vi "4.Open_Select_Profile_Vi.vi"(8 "error in (no error)":errorcluster, 10 "Boolean":bool, 11 "VI Selection":T1=enum."Option window Vi") -> (0 "error out":errorcluster)   [LabVIEW 2021]
uses:
  Control/Vi_selection.ctl
panel:
  out "error in (no error) 2":errorcluster
  out "element":path
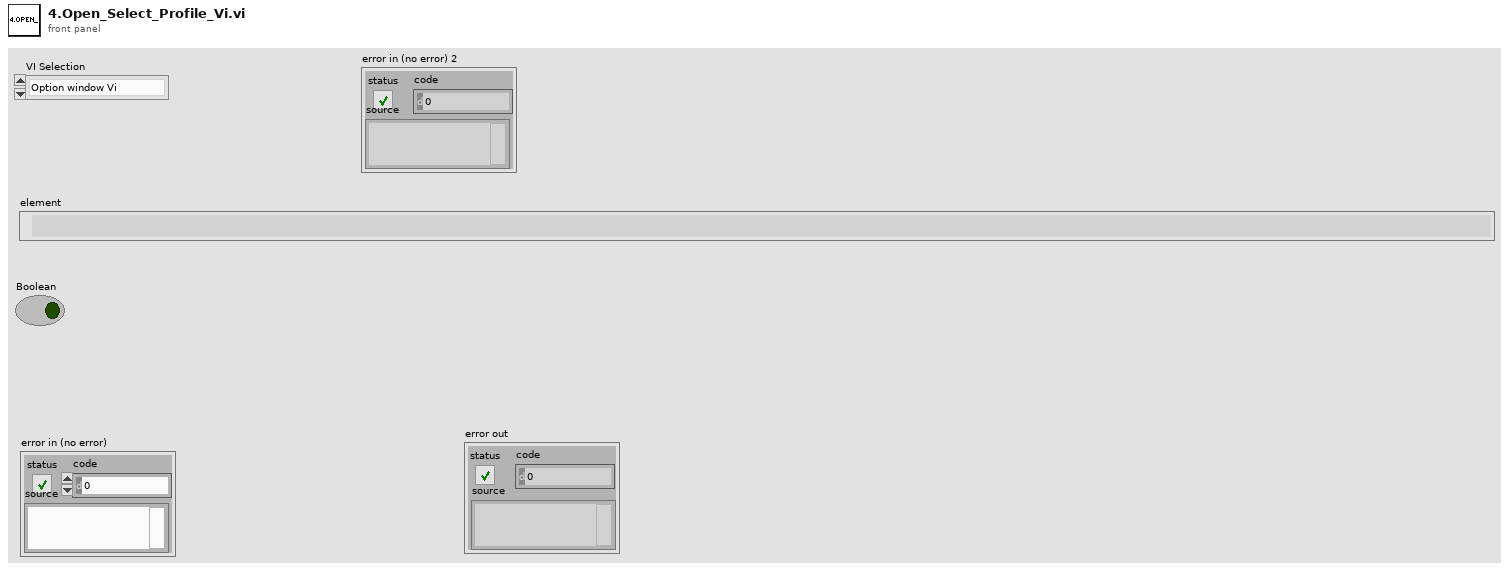
[diagram p1: front panel]
types:
  T1 = typedef "Vi_selection.ctl" = enum16{"Test Editor", "Option window Vi"}
  T2 = enum32{"Invalid", "Standard", "Closed", "Hidden", "Minimized", "Maximized"}
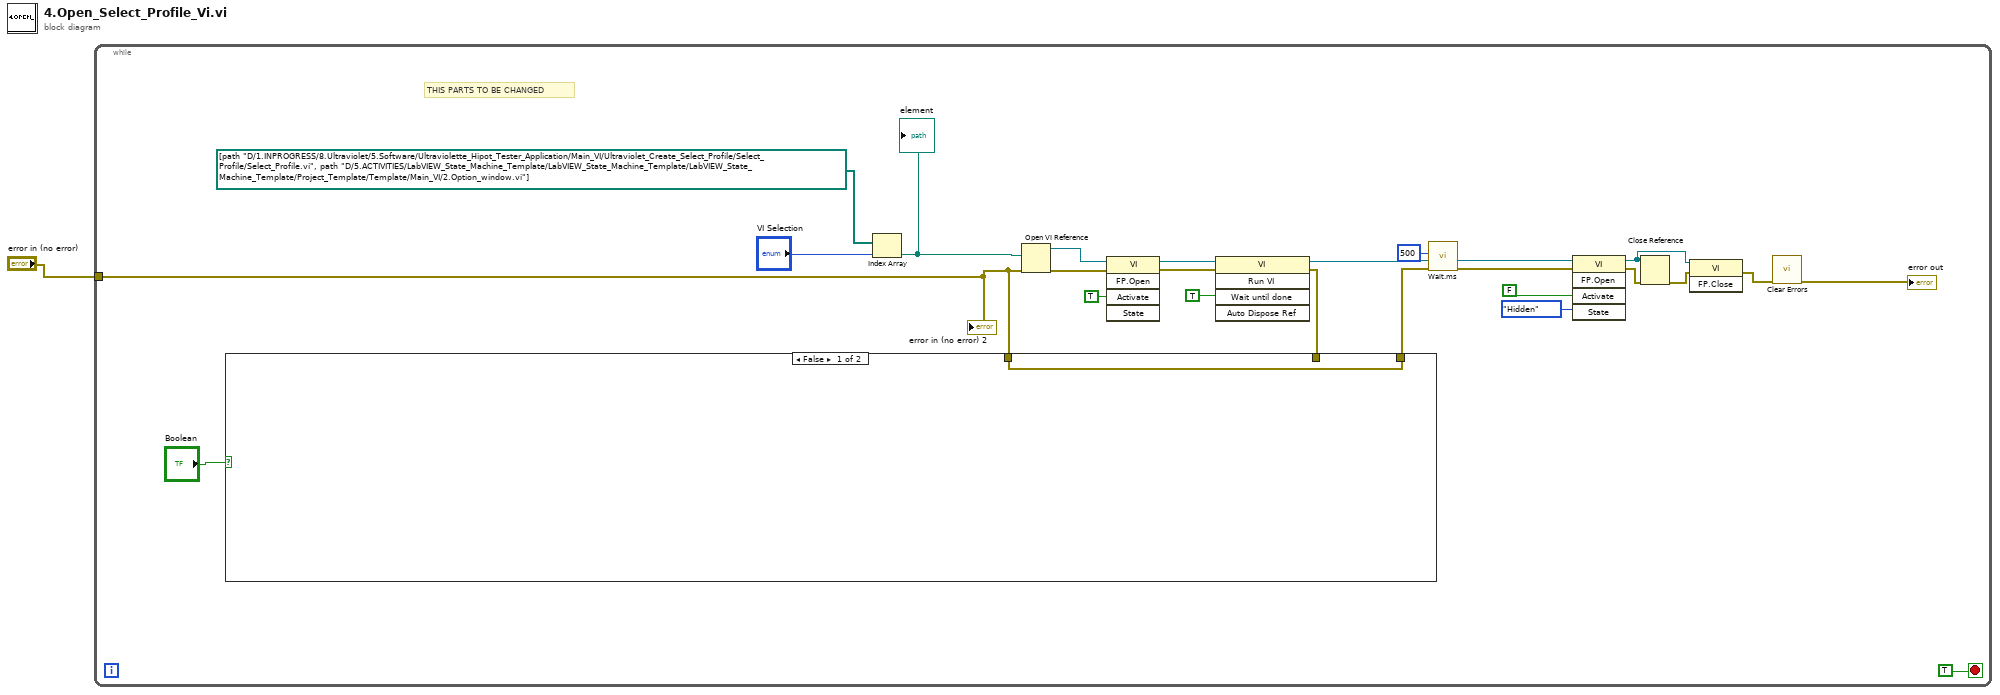
[diagram p0: block diagram]
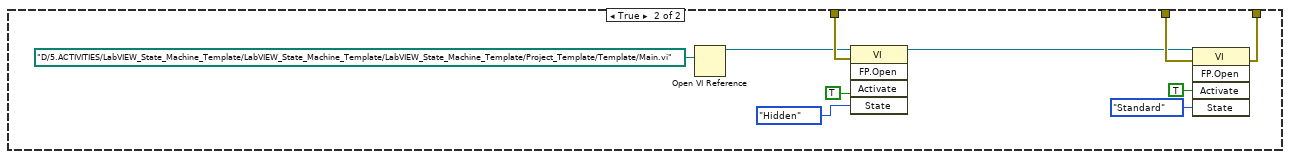
[diagram p2: hidden frame]
diagram:
  n1 = while {
    tunnel: "error in (no error)" -> [w3]
    stop <- TRUE stop-if-true
    # "THIS PARTS TO BE CHANGED"
    n2 = Index Array(array=path[] [path "D:/1.INPROGRESS/8.Ultraviolet/5.Software/Ultraviolette_Hipot_Tester_Application/Main_VI/Ultraviolet_Create_Select_Profile/Select_Profile/Select_Profile.vi", path "D:/5.ACTIVITIES/LabVIEW_State_Machine_Template/LabVIEW_State_Machine_Template/LabVIEW_State_Machine_Template/Project_Template/Template/Main_VI/2.Option_window.vi"], index="VI Selection") -> (element=w2:path)
    "element" <- w2
    n3 = Open VI Reference(vi path=w2, error in (no error)=w3) -> (vi reference=w22:refnum<vi>, error out=w18:errorcluster)  [unwired: 4 in]
    n4 = invoke class="VI" method="FP.Open"(reference=w22, error in=w18, "Activate"=TRUE ("Activate?")) -> (reference out=w20:refnum<vi>, error out=w19:errorcluster)  [unwired: 2 in, 3 out]
    n5 = invoke class="VI" method="Run VI"(reference=w20, error in=w19, "Wait until done"=TRUE ("Wait Until Done")) -> (reference out=w17:refnum<vi>, error out=w13:errorcluster)  [unwired: 2 in, 3 out]
    n6 = case shown="False" "Boolean" {
      tunnel: w3 -> [w26 w33]
      tunnel: w13 -> [_ w29]
      tunnel: [w26 w27] -> w11
      frame False {
      }
      frame True {
        n7 = Open VI Reference(vi path=path "D:/5.ACTIVITIES/LabVIEW_State_Machine_Template/LabVIEW_State_Machine_Template/LabVIEW_State_Machine_Template/Project_Template/Template/Main.vi") -> (vi reference=w32:refnum<vi>)  [unwired: 5 in, 1 out]
        n8 = invoke class="VI" method="FP.Open"(reference=w32, error in=w33, "Activate"=TRUE ("Activate?"), "State"=T2."Hidden") -> (reference out=w28:refnum<vi>)  [unwired: 1 in, 4 out]
        n9 = invoke class="VI" method="FP.Open"(reference=w28, error in=w29, "Activate"=TRUE ("Activate?"), "State"=T2."Standard") -> (error out=w27:errorcluster)  [unwired: 1 in, 4 out]
      }
    }
    n10 = call "Wait.ms.vi"("error in"=w11, "milliseconds to wait"=u32 500) -> ("error out"=w12:errorcluster)  [unwired: 9 in]
    n11 = invoke class="VI" method="FP.Open"(reference=w17, error in=w12, "Activate"=FALSE ("Activate?"), "State"=T2."Hidden") -> (reference out=w6:refnum<vi>, error out=w16:errorcluster)  [unwired: 1 in, 3 out]
    n12 = Close Reference(reference=w6, error in (no error)=w16) -> (error out=w7:errorcluster)
    n13 = invoke class="VI" method="FP.Close"(reference=w6, error in=w7) -> (error out=w8:errorcluster)  [unwired: 1 in, 2 out]
    n14 = call <vilib>:"Clear Errors.vi"("error in (no error)"=w8) -> ("error out"=→"error out":errorcluster)  [unwired: 5 in, 1 out]
    "error in (no error) 2" <- w3
  }
